vi "configure runtime data.vi"(4 "output dictionary":refnum<class "data dictionary.lvclass">, 6 "input dictionary":refnum<class "data dictionary.lvclass">, 8 "error in":errorcluster, 10 "Slave Info List":T6(array[cluster]), 11 "Profibus Module configuration in":refnum<class "Profibus Module configuration.lvclass">) -> (0 "error out":errorcluster, 1 "diagnostics":T1[](array[typedef]), 2 "inputs":T3[](array[typedef]), 3 "outputs":T3[](array[typedef]), 5 "full command list":u32[](array[numeric]))   [LabVIEW 2013, in "Profibus Module runtime.lvclass"]
uses:
  Profibus Module runtime.lvclass
  configuration/Profibus Module configuration.lvclass
  profibus slave configuration.ctl
  profibus mapping configuration.ctl
  <vilib>/NI/Tag Bus/tag/Data Type.ctl
  <vilib>/NI/Tag Bus/dictionary/data dictionary.lvclass
  profibus diagnostics reporting.ctl
  configuration/error throw specification.ctl
  configuration/Profibus Module configuration.lvclass/Profibus Module configuration.ctl
  dynamic profibus/profibus master action.ctl
  <vilib>/NI/Tag Bus/tag/tag descriptor.lvclass/tag descriptor.ctl
  <vilib>/NI/Tag Bus/dictionary/data dictionary.lvclass/data dictionary.ctl
  configuration/Read slave diagnostics.vi
  <vilib>/NI/Tag Bus/dictionary/look up tag by type.vi
  <vilib>/NI/Tag Bus/dictionary/lookup polymorphs/locate Array of U8.vi
  <vilib>/NI/Tag Bus/tag/read tag name.vi
  <vilib>/NI/Tag Bus/dictionary/search/find data index.vi
  <vilib>/NI/Tag Bus/dictionary/search/search string list.vi
  <vilib>/NI/Tag Bus/dictionary/tag not found.vi
  dynamic profibus/dynamic profibus.lvlib
  <vilib>/NI/Tag Bus/tag/tag descriptor.lvclass
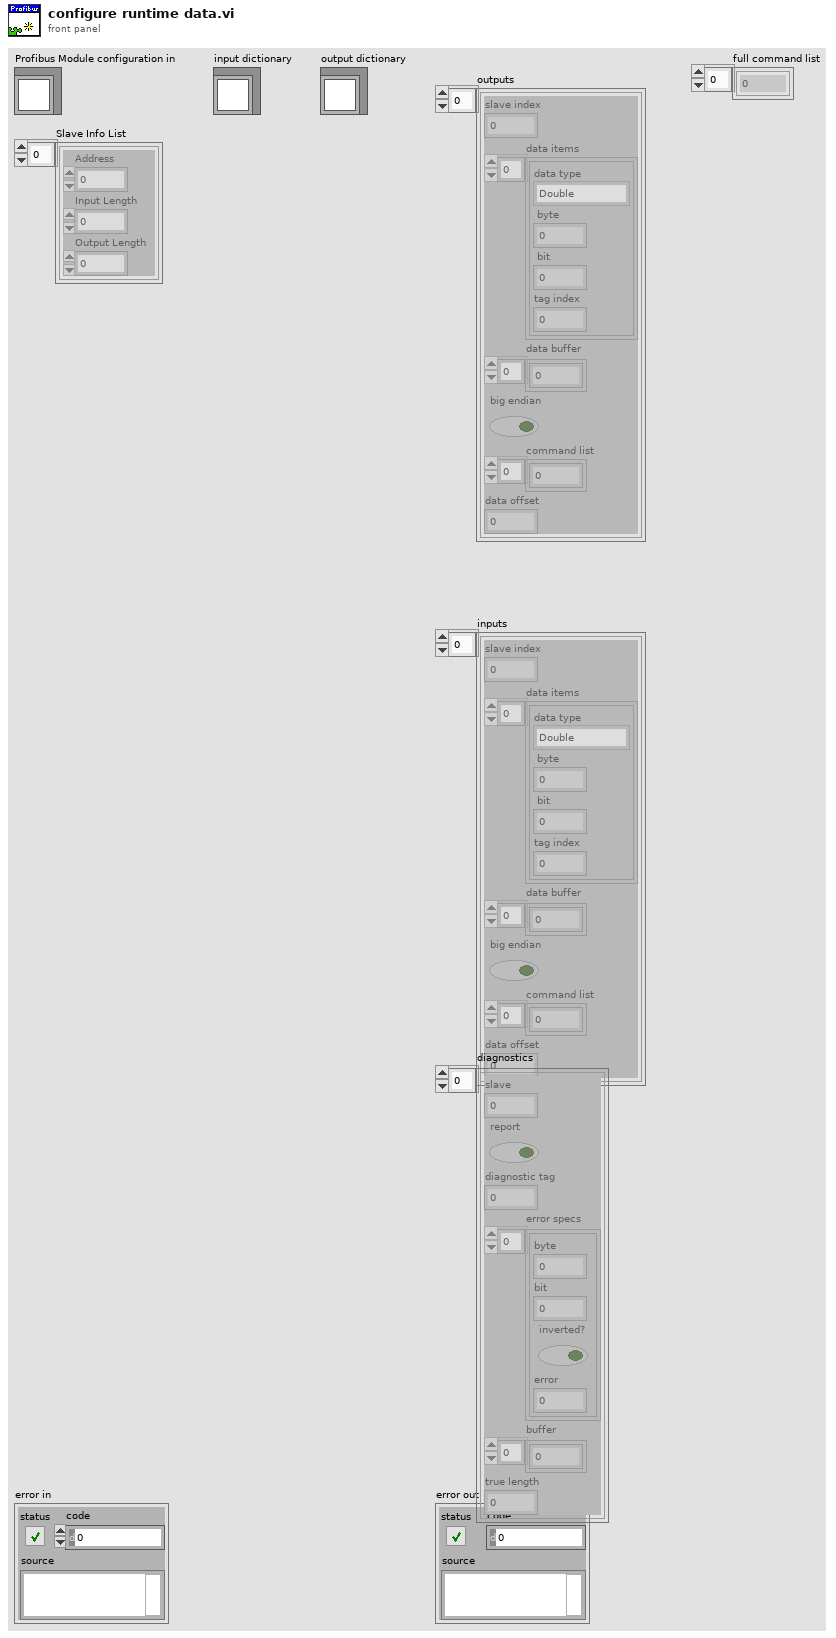
[diagram p1: front panel]
types:
  T1 = typedef "Profibus Module runtime.lvclass/profibus diagnostics reporting.ctl" = cluster{"slave":i8, "report":bool, "diagnostic tag":i32, "error specs":T2[], "buffer":u8[], "true length":u8}
  T2 = typedef "Profibus Module configuration.lvclass/error throw specification.ctl" = cluster{"byte":i32, "bit":i32, "inverted?":bool, "error":i32}
  T3 = typedef "Profibus Module runtime.lvclass/profibus slave configuration.ctl" = cluster{"slave index":i8, "data items":T4[], "data buffer":u8[], "big endian":bool, "command list":u32[], "data offset":u8}
  T4 = typedef "Profibus Module runtime.lvclass/profibus mapping configuration.ctl" = cluster{"data type":T5, " byte":i32, " bit":i32, "tag index":i32}
  T5 = typedef "tag bus.lvlib/tag descriptor.lvclass/Data Type.ctl" = enum16{"Double", "Single", "I64", "I32", "I16", "I8", "U64", "U32", "U16", "U8", "Boolean", "String", "Array of Double", "Array of Single", "Array of I64", "Array of I32", "Array of I16", "Array of I8", "Array of U64", "Array of U32", "Array of U16", "Array of U8", "Array of Boolean", "Array of String"}
  T6 = cluster{"Address":i8, "Input Length":u8, "Output Length":u8}[]
  T7 = typedef "dynamic profibus.lvlib/profibus master action.ctl" = enum8{"initialize", "uninitialize", "stop", "get input", "get input size", "set output", "get output size", "get diagnostic", "transfer data", "transfer diagnostics", "read many inputs"}
  T8 = typedef "Profibus Module configuration.lvclass/endianness setting.ctl" = cluster{"slave":i8, "big endian":bool}
  T9 = typedef "Profibus Module runtime.lvclass/required data sets.ctl" = cluster{"Address":i8, "Input Start":u8, "Input End":u8, "Output Start":u8, "Output End":u8, "chan in":refnum<class "Profibus channel.lvclass">[], "chan out":refnum<class "Profibus channel.lvclass">[]}
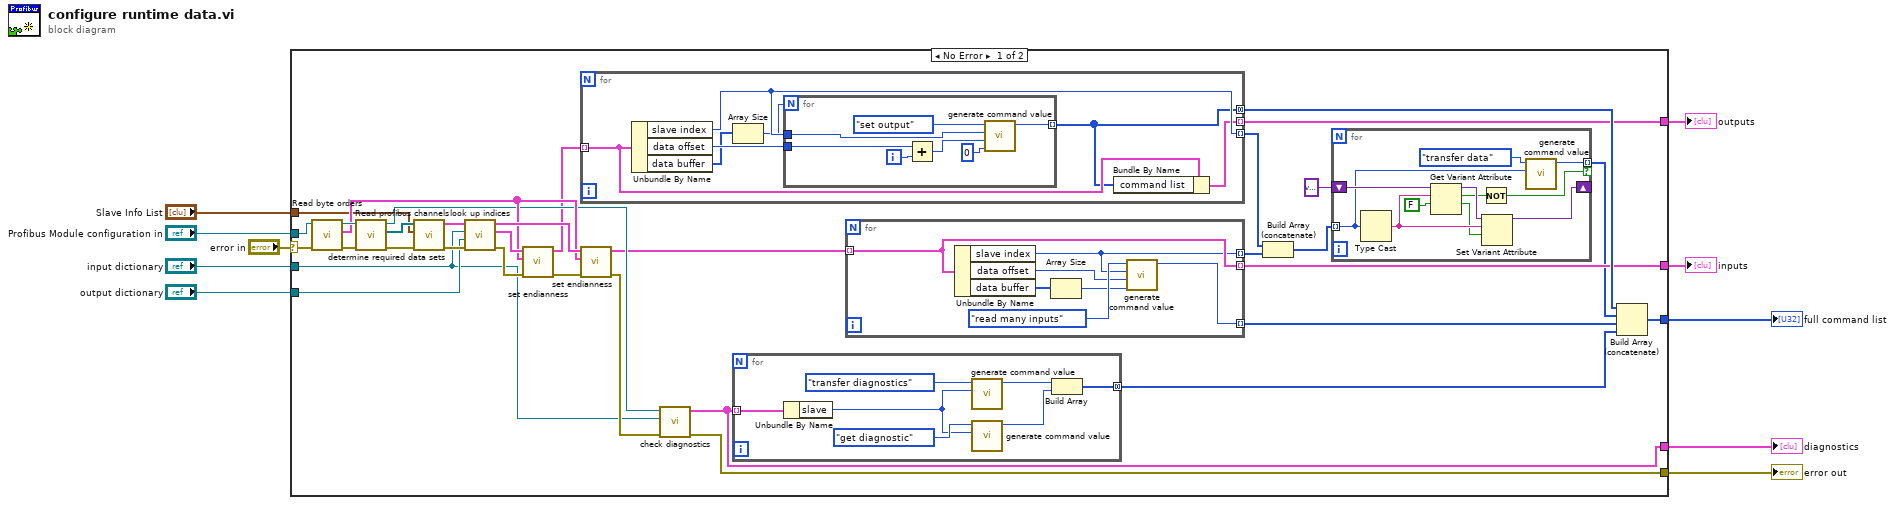
[diagram p0: block diagram]
diagram:
  n1 = case shown="No Error" "error in" {
    selector: "error in" -> [w11 w83]
    tunnel: "Profibus Module configuration in" -> [w41 _]
    tunnel: [w36 w83] -> w9
    tunnel: [w33 _] -> w8
    tunnel: [w25 _] -> w7
    tunnel: [w24 _] -> w6
    tunnel: "Slave Info List" -> [w20 _]
    tunnel: "output dictionary" -> [w16 _]
    tunnel: "input dictionary" -> [w15 _]
    tunnel: [w12 _] -> w2
    frame No Error {
      n2 = call "Read byte orders.vi"("error in"=w11, "Profibus Module configuration in"=w41) -> ("error out"=w39:errorcluster, "byte orders"=w37:T8[], "Profibus Module configuration out"=w40:refnum<class "Profibus Module configuration.lvclass">)  [unwired: 7 in]
      n3 = call "Read profibus channels.vi"("error in"=w39, "Profibus Module configuration in"=w40) -> ("error out"=w22:errorcluster, "channels"=w21:refnum<class "Profibus channel.lvclass">[], "Profibus Module configuration out"=w34:refnum<class "Profibus Module configuration.lvclass">)  [unwired: 7 in]
      n4 = call "determine required data sets.vi"("error in"=w22, "Slave Info List"=w20, "channels"=w21) -> ("error out"=w18:errorcluster, "slave data subsets"=w17:T9[])  [unwired: 7 in]
      n5 = call "look up indices.vi"("error in"=w18, "output dictionary"=w16, "input dictionary"=w15, "slave data subsets"=w17) -> ("error out"=w19:errorcluster, "outputs"=w42:T3[], "inputs"=w43:T3[])  [unwired: 5 in]
      n6 = call "set endianness.vi"("error in"=w19, "byte orders"=w37, "config in"=w42) -> ("error out"=w38:errorcluster, "config out"=w31:T3[])  [unwired: 7 in]
      n7 = for {
        tunnel: w31 -> [w60] mode=indexing
        tunnel: [w59] -> w27 mode=concatenating
        tunnel: [w61] -> w29 mode=indexing
        tunnel: [w58] -> w25 mode=indexing
        n8 = Unbundle By Name(w60) -> ("slave index"=w61:i8, "data offset"=w57:u8, "data buffer"=w56:u8[])
        n9 = Array Size(array=w56) -> (size(s)=w55:i32)
        n10 = for {
          N: w55 -> [_]
          tunnel: [w68] -> w59 mode=indexing
          tunnel: w61 -> [w66]
          tunnel: w57 -> [w62]
          i -> [w65]
          n11 = Add(x=w62, y=w65) -> (x+y=w63:i32)
          n12 = call "generate command value.vi"("data"=u8 0, "index"=w63, "device"=w66, "action"=profibus_master_action."set output") -> ("Element"=w68:u32)  [unwired: 7 in]
        }
        n13 = Bundle By Name(cluster=w60, "command list"=w59) -> (w58:T3)
      }
      n14 = call "set endianness.vi"("error in"=w38, "byte orders"=w37, "config in"=w43) -> ("error out"=w35:errorcluster, "config out"=w32:T3[])  [unwired: 7 in]
      n15 = call "check diagnostics.vi"("error in"=w35, "data dictionary in"=w15, "Profibus Module configuration in"=w34) -> ("error out"=w36:errorcluster, "diagnostics"=w33:T1[])  [unwired: 7 in]
      n16 = for {
        tunnel: w33 -> [w82] mode=indexing
        tunnel: [w79] -> w13 mode=concatenating
        n17 = Unbundle By Name(w82) -> ("slave"=w76:i8)
        n18 = call "generate command value.vi"("device"=w76, "action"=profibus_master_action."transfer diagnostics") -> ("Element"=w80:u32)  [unwired: 9 in]
        n19 = call "generate command value.vi"("device"=w76, "action"=profibus_master_action."get diagnostic") -> ("Element"=w81:u32)  [unwired: 9 in]
        n20 = Build Array(w80, w81) -> (w79:u32[])
      }
      n21 = for {
        tunnel: w32 -> [w75] mode=indexing
        tunnel: [w74] -> w28 mode=indexing
        tunnel: [w72] -> w30 mode=indexing
        tunnel: [w75] -> w24 mode=indexing
        n22 = Unbundle By Name(w75) -> ("slave index"=w72:i8, "data offset"=w71:u8, "data buffer"=w70:u8[])
        n23 = Array Size(array=w70) -> (size(s)=w69:i32)
        n24 = call "generate command value.vi"("data"=w69, "index"=w71, "device"=w72, "action"=profibus_master_action."read many inputs") -> ("Element"=w74:u32)  [unwired: 7 in]
      }
      n25 = Build Array (concatenate)(w29, w30) -> (w26:i8[])
      n26 = for {
        tunnel: [w46] -> w14 mode=indexing if=w48
        tunnel: w26 -> [w44] mode=indexing
        shift-right: [w54] -> _
        shift-left: variant -> [w53]
        n27 = Type Cast(x=w44) -> (*(type *) &x=w51:string)  [unwired: 1 in]
        n28 = Get Variant Attribute(Variant=w53, name=w51, default value (empty Variant)=FALSE) -> (duplicate Variant=w52:variant, found=w49:bool, value=w47:bool)  [unwired: 1 in, 1 out]
        n29 = Not(x=w49) -> (.not. x?=w48:bool)
        n30 = Set Variant Attribute(Variant=w52, name=w51, value=w47) -> (Variant out=w54:variant)  [unwired: 1 in, 2 out]
        n31 = call "generate command value.vi"("device"=w44, "action"=profibus_master_action."transfer data") -> ("Element"=w46:u32)  [unwired: 9 in]
      }
      n32 = Build Array (concatenate)(w27, w14, w28, w13) -> (w12:u32[])
    }
    frame Error {
    }
  }
  "error out" <- w9
  "diagnostics" <- w8
  "outputs" <- w7
  "inputs" <- w6
  "full command list" <- w2
